vi "[ex ce]_Array - Creating numeric sequences.vi"() -> ()   [LabVIEW 2021]
doc: "<B>Creating numeric sequences in a script</B>\n\nThe VI demonstrates a use of some functions to build 1D arrays with numeric sequences.\n\n::: CalcExpress Toolkit :::\nCopyright (c) 2000-2026 Konstantin Shifershteyn. All rights reserved."
panel:
  out "AR3":dbl[](array[numeric])
  out "AR1":dbl[](array[numeric])
  in  "Expression":string="init  = 1;\nfinal = 10;\nstep  = 3;\nnum   = 10;\n\nAR1 = nvecifn(init, final, num);\nAR2 = nvecifs(init, final, step);\nAR3 = nvecins(init, num ,  step);\n"
  out "AR2":dbl[](array[numeric])
  # "resulting arrays"
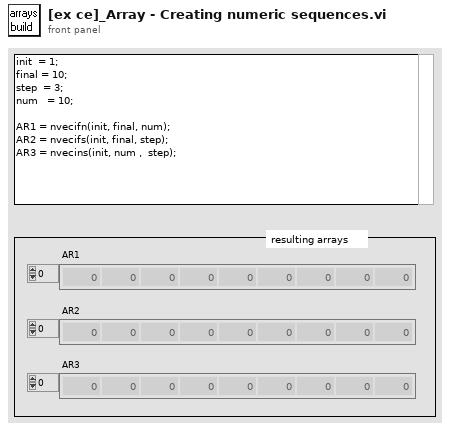
[diagram p1: front panel]
types:
  T1 = typedef "VarMan Variable Context Handle.ctl" = i32
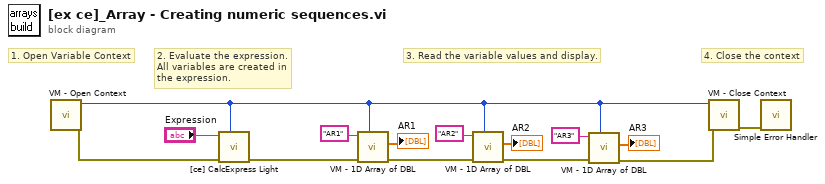
[diagram p0: block diagram]
diagram:
  # "4. Close the context"
  # "3. Read the variable values and display."
  # "2. Evaluate the expression.\nAll variables are created in\nthe expression."
  # "1. Open Variable Context"
  n1 = call "VM - Open Context.vi"() -> ("error out"=w9:errorcluster, "VC Handle out"=w1:T1)  [unwired: 9 in, 1 out]
  n2 = call "[ce] CalcExpress Light.vi"("VC Handle"=w1, "error in"=w9, "expression"="Expression") -> ("error out"=w7:errorcluster)  [unwired: 6 in, 2 out]
  n3 = call "VM - 1D Array of DBL.vi"("VC Handle"=w1, "error in"=w7, "name_spec"="AR1" ("name in")) -> ("error out"=w4:errorcluster, "value out"=→"AR1":dbl[])  [unwired: 3 in, 4 out]
  n4 = call "VM - 1D Array of DBL.vi"("VC Handle"=w1, "error in"=w4, "name_spec"="AR2" ("name in")) -> ("error out"=w3:errorcluster, "value out"=→"AR2":dbl[])  [unwired: 3 in, 4 out]
  n5 = call "VM - 1D Array of DBL.vi"("VC Handle"=w1, "error in"=w3, "name_spec"="AR3" ("name in")) -> ("error out"=w2:errorcluster, "value out"=→"AR3":dbl[])  [unwired: 3 in, 4 out]
  n6 = call "VM - Close Context.vi"("error in"=w2, "VC Handle"=w1) -> ("error out"=w8:errorcluster)  [unwired: 8 in, 1 out]
  n7 = call <vilib>:"Simple Error Handler.vi"("error in (no error)"=w8) -> ()  [unwired: 4 in, 5 out]
